vi "fake tool required input.vi"(10 "b":i32, 11 "a":i32) -> (3 "a*b":i32)   [LabVIEW 2020, in "MCP Server tests.lvlib"]
doc: "This is a fake tool to test the MCP server toolkit. It multiplies its two inputs a and b, which are both required."
uses:
  MCP Server tests.lvlib
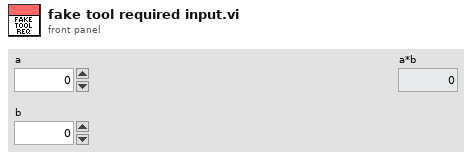
[diagram p1: front panel]
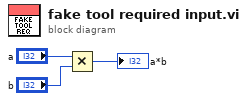
[diagram p0: block diagram]
diagram:
  n1 = Multiply(x="a", y="b") -> (x*y=→"a*b":i32)
